vi "FCC U-NII1 BE Integration Method.vi"(8 "error in (no error)":errorcluster, 11 "Band Edge in":refnum<class "Band Edge.lvclass">) -> (0 "error out":errorcluster, 3 "Band Edge out":refnum<class "Band Edge.lvclass">)   [LabVIEW 2023, in "Spectrum Analyzer.lvlib" / "Band Edge.lvclass"]
uses:
  Band Edge.lvclass
  FSV-40N/FSV-40N.lvclass
  D:/Project/IST008_FCC Band Edge Measurement/IST008-FCC-Band-Edge/src/Spectrum Analyzer/Interface_Spectrum/Interface_Spectrum.lvclass
  TYPE DEFINITION/TYPE FCC Part15c Integration BandEdge Setting Cluster.ctl
  TYPE DEFINITION/TYPE Spectrum Window Select.ctl
  TYPE DEFINITION/TYPE Start and Stop Frequency.ctl
  TYPE DEFINITION/TYPE Display Trace Mode Select.ctl
  TYPE DEFINITION/TYPE Detect Mode Select.ctl
  TYPE DEFINITION/TYPE ACLR Setting Param.ctl
  TYPE DEFINITION/TYPE Center and Span Frequency.ctl
  TYPE DEFINITION/TYPE Frequency Line Param.ctl
  FSV-40N/FSV-40N.lvclass/FSV-40N.ctl
  Band Edge.lvclass/Band Edge.ctl
  Spectrum Analyzer.lvlib
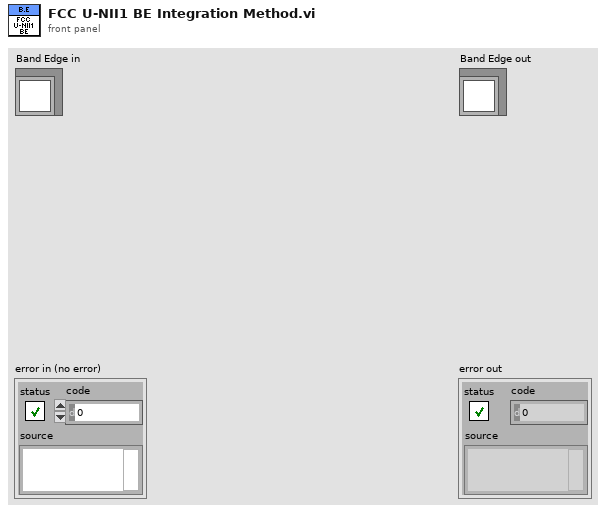
[diagram p1: front panel]
types:
  T1 = typedef "Spectrum Analyzer.lvlib/TYPE FCC Part15c Integration BandEdge Setting Cluster.ctl" = cluster{"Window":T2, "Start/Stop Frequency(Hz)":T3, "Ref":dbl, "Atten":i32, "RBW(Hz)":dbl, "VBW(Hz)":dbl, "Sweep Time(sec)":dbl, "Sweep Time Auto?":bool, "Sweep Count":u32, "Sweep Point":u32, "Trace/Det":cluster{"Trace Mode":T4, "Detector Type":T5}[], "ACLR Param":T6, "Center and Span Frequency(Hz)":T7, "Frequency Line (Hz)":T8}
  T2 = typedef "Spectrum Analyzer.lvlib/TYPE Spectrum Window Select.ctl" = enum16{"Spectrum 1", "Spectrum 2", "Spectrum 3", "Spectrum 4"}
  T3 = typedef "Spectrum Analyzer.lvlib/TYPE Start and Stop Frequency.ctl" = cluster{"Start":dbl, "Stop":dbl}
  T4 = typedef "Spectrum Analyzer.lvlib/TYPE Display Trace Mode Select.ctl" = enum16{"Clear Write", "Max Hold", "Min Hold", "Average", "View"}
  T5 = typedef "Spectrum Analyzer.lvlib/TYPE Detect Mode Select.ctl" = enum16{"Det Auto", "Auto Peak", "Positive Peak", "Negative Peak", "Sample", "RMS", "Average", "Quasipeak", "CISPR Average", "RMS Average"}
  T6 = typedef "Spectrum Analyzer.lvlib/TYPE ACLR Setting Param.ctl" = cluster{"Bandwidth":dbl, "Offset":dbl, "Tx Channel Count":i32}
  T7 = typedef "Spectrum Analyzer.lvlib/TYPE Center and Span Frequency.ctl" = cluster{"Center":dbl, "Span":dbl}
  T8 = typedef "Spectrum Analyzer.lvlib/TYPE Frequency Line Param.ctl" = cluster{"Line 1":dbl, "Line 2":dbl, "Activate Line1?":bool, "Activate Line2?":bool}
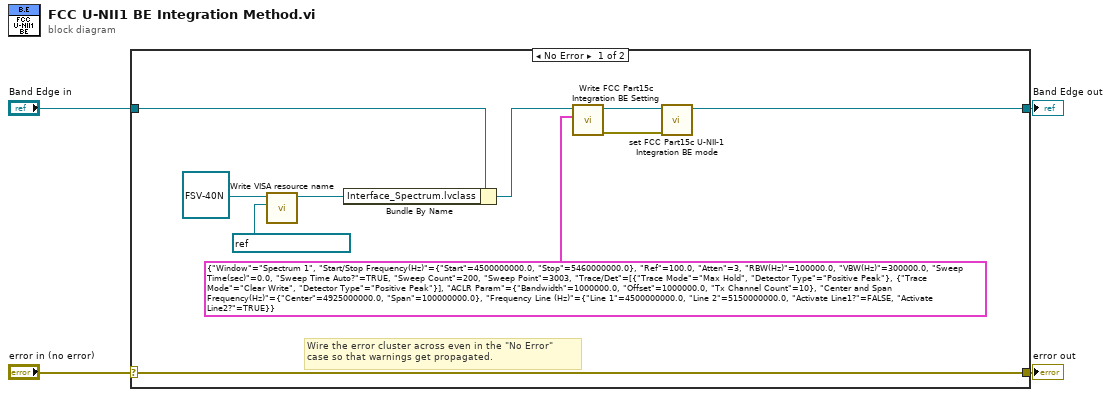
[diagram p0: block diagram]
diagram:
  n1 = case shown="No Error" "error in (no error)" {
    selector: "error in (no error)" -> [w14 w16]
    tunnel: [w14 w16] -> w3
    tunnel: [w8 w15] -> w1
    tunnel: "Band Edge in" -> [w10 w15]
    frame No Error {
      # "Wire the error cluster across even in the \"No Error\"\ncase so that warnings get propagated."
      n2 = call "Write VISA resource name.vi"("VISA resource name"=refnum<visa-resource-name> "GPIB0::18::INSTR", "FSV-40N in"=refnum<class "FSV-40N.lvclass"> refnum ("Spectrum Analyzer.lvlib:FSV-40N.lvclass")) -> ("FSV-40N out"=w11:refnum<class "FSV-40N.lvclass">)  [unwired: 8 in, 1 out]
      n3 = Bundle By Name(cluster=w10, "Interface_Spectrum.lvclass"=w11) -> (w9:refnum<class "Band Edge.lvclass">)
      n4 = call "Write FCC Part15c Integration BE Setting.vi"("Cluster"=T1 {"Window"=enum."Spectrum 1", "Start/Stop Frequency(Hz)"={"Start"=4500000000.0, "Stop"=5460000000.0}, "Ref"=100.0, "Atten"=3, "RBW(Hz)"=100000.0, "VBW(Hz)"=300000.0, "Sweep Time(sec)"=0.0, "Sweep Time Auto?"=TRUE, "Sweep Count"=200, "Sweep Point"=3003, "Trace/Det"=[{"Trace Mode"=enum."Max Hold", "Detector Type"=enum."Positive Peak"}, {"Trace Mode"=enum."Clear Write", "Detector Type"=enum."Positive Peak"}], "ACLR Param"={"Bandwidth"=1000000.0, "Offset"=1000000.0, "Tx Channel Count"=10}, "Center and Span Frequency(Hz)"={"Center"=4925000000.0, "Span"=100000000.0}, "Frequency Line (Hz)"={"Line 1"=4500000000.0, "Line 2"=5150000000.0, "Activate Line1?"=FALSE, "Activate Line2?"=TRUE}}, "Band Edge in"=w9) -> ("error out"=w5:errorcluster, "Band Edge out"=w7:refnum<class "Band Edge.lvclass">)  [unwired: 8 in]
      n5 = call "set FCC Part15c U-NII-1 Integration BE mode.vi"("error in (no error)"=w5, "Band Edge in"=w7) -> ("Band Edge out"=w8:refnum<class "Band Edge.lvclass">)  [unwired: 8 in, 1 out]
    }
    frame Error {
    }
  }
  "error out" <- w3
  "Band Edge out" <- w1
